vi "PathPlanner_Path_ConstTargetSpacing.vi"() -> (3 "TargetSpacing":dbl=0.2)   [LabVIEW 2019, in "PathPlanner24.lvlib"]
doc: "Constant - TargetSpacing\n\nInputs: \n - <none>\n\nOutputs:\n - TargetSpacing - double - constant"
uses:
  PathPlanner24.lvlib
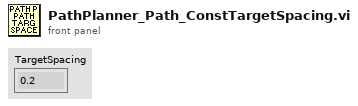
[diagram p1: front panel]
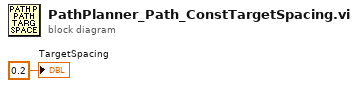
[diagram p0: block diagram]
diagram:
  "TargetSpacing" <- 0.2 ("TargetIncrement")
